vi "VIH Project Tree - Relink Invalid Files in a Menu Hierarchy.vi"(8 "error in":errorcluster, 9 "old Item Path":path, 10 "new Item Path":path, 11 "Project Tree":T1) -> (0 "error out":errorcluster, 3 "dup Project Tree":T1)   [LabVIEW 2014]
doc: "::: VI Helpeks :::\nCopyright (c) 2000-2026 Konstantin Shifershteyn. All rights reserved."
uses:
  VIH Project Tree Typedef - Tree Refnum.ctl
  _VIH HelpGen - Palette.llb/VIH HelpGen Typedef - Palette - Item Type Enum.ctl
panel:
  # "VI Helpeks\nCopyright (c) 2012-2026 Konstantin Shifershteyn"
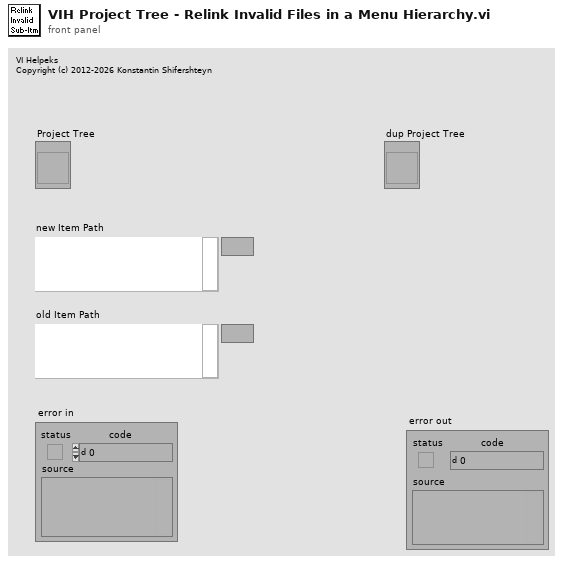
[diagram p1: front panel]
types:
  T1 = typedef "VIH Project Tree Typedef - Tree Refnum.ctl" = refnum<vi>
  T2 = typedef "VIH HelpGen Typedef - Palette - Item Type Enum.ctl" = enum32{"<Invalid>", "<unknown>", "VI", "Menu", "LV Func", "Express VI", "Poly VI", "CTL", "HTML"}
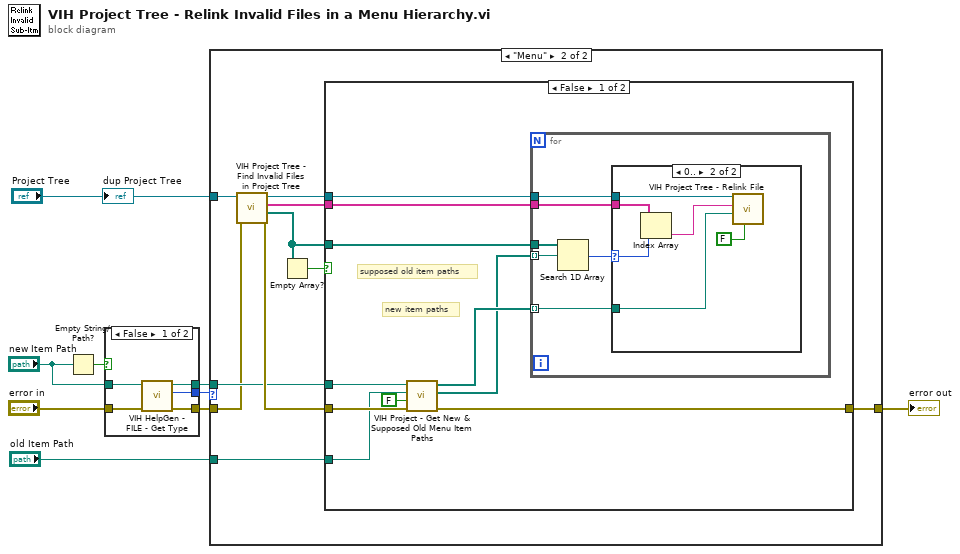
[diagram p0: block diagram]
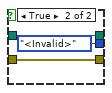
[diagram p2: hidden frame]
diagram:
  n1 = Empty String/Path?(string/path="new Item Path") -> (empty?=w2:bool)
  n2 = case shown="False" w2 {
    tunnel: [w14 w17] -> w6
    tunnel: "new Item Path" -> [w13 w17]
    tunnel: "error in" -> [w12 w16]
    tunnel: [w11 w16] -> w4
    tunnel: [w10 VIH_HelpGen_Typedef_-_Palette_-_Item_Type_Enum."<Invalid>" ("File Type")] -> w3
    frame False {
      n3 = call "VIH HelpGen - FILE - Get Type.vi"("error in"=w12, "File Path"=w13) -> ("error out"=w11:errorcluster, "File Type"=w10:T2, "dup File Path"=w14:path)  [unwired: 7 in]
    }
    frame True {
    }
  }
  n4 = case shown="\"Menu\"" w3 {
    tunnel: [w18 w28] -> w9
    tunnel: "old Item Path" -> [_ w27]
    tunnel: "Project Tree" -> [_ w26]
    tunnel: w6 -> [_ w20]
    tunnel: w4 -> [w18 w19]
    frame Default {
    }
    frame "Menu" {
      n5 = call "VIH Project Tree - Find Invalid Files in Project Tree.vi"("error in"=w19, "Project Tree"=w26) -> ("error out"=w23:errorcluster, "Item Paths"=w24:path[], "Tree Item Tags"=w21:string[], "dup Project Tree"=w22:T1)  [unwired: 6 in]
      n6 = Empty Array?(array=w24) -> (empty?=w25:bool)
      n7 = case shown="False" w25 {
        tunnel: w20 -> [w37 _]
        tunnel: w23 -> [w36 w51]
        tunnel: [w35 w51] -> w28
        tunnel: w24 -> [w38 _]
        tunnel: w27 -> [w34 _]
        tunnel: w22 -> [w30 _]
        tunnel: w21 -> [w29 _]
        frame False {
          # "new item paths"
          # "supposed old item paths"
          n8 = call "VIH Project - Get New & Supposed Old Menu Item Paths.vi"("error in"=w36, "Test File Type (T)"=FALSE, "old Menu Path"=w34, "new Menu Path"=w37) -> ("error out"=w35:errorcluster, "Supposed Old Item Paths"=w31:path[], "New Item Paths"=w32:path[])  [unwired: 5 in]
          n9 = for {
            tunnel: w32 -> [w42] mode=indexing
            tunnel: w38 -> [w44]
            tunnel: w31 -> [w41] mode=indexing
            tunnel: w30 -> [w40]
            tunnel: w29 -> [w39]
            n10 = Search 1D Array(1D array=w44, element=w41) -> (index of element=w43:i32)  [unwired: 1 in]
            n11 = case shown="0.." w43 {
              selector: w43 -> [_ w48]
              tunnel: w42 -> [_ w46]
              tunnel: w40 -> [_ w50]
              tunnel: w39 -> [_ w49]
              frame ..-1 {
              }
              frame 0.. {
                n12 = Index Array(array=w49, index=w48) -> (element=w47:string)
                n13 = call "VIH Project Tree - Relink File.vi"("Ena Dialog Message (T)"=FALSE, "New File Path"=w46, "Tree Item Tag"=w47, "Project Tree"=w50) -> ()  [unwired: 4 in, 4 out]
              }
            }
          }
        }
        frame True {
        }
      }
    }
  }
  "error out" <- w9
  "dup Project Tree" <- "Project Tree"
